vi "Launcher.vi"() -> ()   [LabVIEW 2024]
uses:
  Libraries/Mysterious DQMH Module/Mysterious DQMH Module.lvlib
panel:
  out "Button Pressed":enum16{"Yes", "No", "Maybe"}(ring)
  in  "Message to Display":string
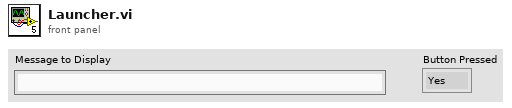
[diagram p1: front panel]
types:
  T1 = typedef "Mysterious DQMH Module.lvlib/Broadcast Events--cluster.ctl" = cluster{"Module Did Init":refnum<user-event>, "Status Updated":refnum<user-event>, "Error Reported":refnum<user-event>, "Module Did Stop":refnum<user-event>, "Update Module Execution Status":refnum<user-event>, "Button was Pressed":refnum<user-event>}
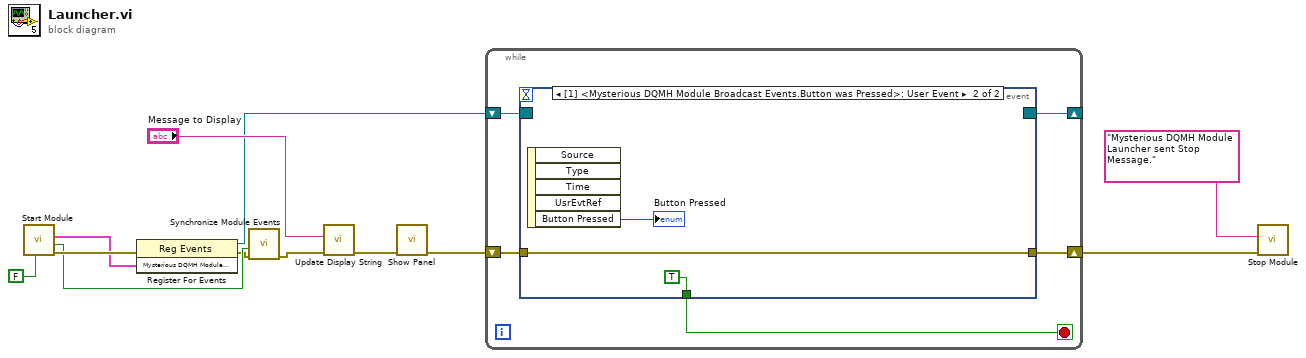
[diagram p0: block diagram]
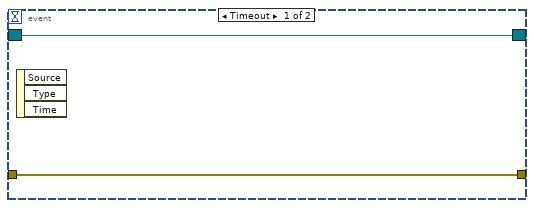
[diagram p2: hidden frame]
diagram:
  n1 = call "Start Module.vi"("Show Main VI Diagram on Init (F)"=FALSE) -> ("error out"=w12:errorcluster, "Wait for Event Sync?"=w11:bool, "Mysterious DQMH Module Broadcast Events"=w10:T1)  [unwired: 6 in, 2 out]
  n2 = register-events(error in=w12, w10) -> (reference out=w5:refnum<event-registration>, error out=w1:errorcluster)  [unwired: 1 in]
  n3 = call "Synchronize Module Events.vi"("error in"=w1, "Wait for Event Sync?"=w11) -> ("error out"=w3:errorcluster)  [unwired: 9 in]
  n4 = call "Update Display String.vi"("error in"=w3, "Message to Display"="Message to Display") -> ("error out"=w6:errorcluster)  [unwired: 9 in]
  n5 = call "Show Panel.vi"("error in"=w6) -> ("error out"=w2:errorcluster)  [unwired: 10 in]
  n6 = while {
    shift-right: [w16] -> w4
    shift-left: w2 -> [w17]
    shift-right: [w14] -> _
    shift-left: w5 -> [w15]
    stop <- w13 stop-if-true
    n7 = event shown="[1] <Mysterious DQMH Module Broadcast Events.Button was Pressed>: User Event" {
      selector: w15 -> [w18 _]
      dyn-events: [w18 _] -> w14
      timeout: _ -> [_ _]
      tunnel: w17 -> [w19 w21]
      tunnel: [w19 w21] -> w16
      tunnel: [_ TRUE] -> w13
      event Timeout {
        n8 = event-data() -> ()  [unwired: 1 in, 3 out]
      }
      event User Event {
        n9 = event-data() -> ("Button Pressed"=→"Button Pressed":enum16{"Yes", "No", "Maybe"})  [unwired: 1 in, 4 out]
      }
    }
  }
  n10 = call "Stop Module.vi"("error in"=w4, "Origin"="Mysterious DQMH Module Launcher sent Stop Message.") -> ()  [unwired: 9 in, 1 out]
